vi "Main_CLIWrapper.vi"(11 "Inputs":string[](array[string])) -> (2 "Output/Failure":string, 3 "CLI Process Return Code":i32)   [LabVIEW 2019]
uses:
  <vilib>/Utility/error.llb/DialogType.ctl
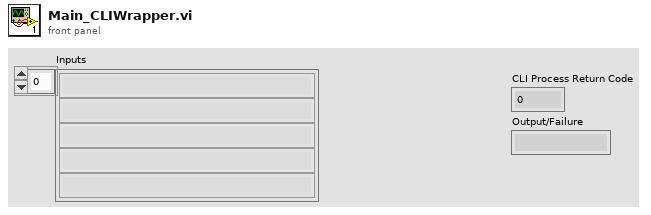
[diagram p1: front panel]
types:
  T1 = typedef "DialogType.ctl" = u16
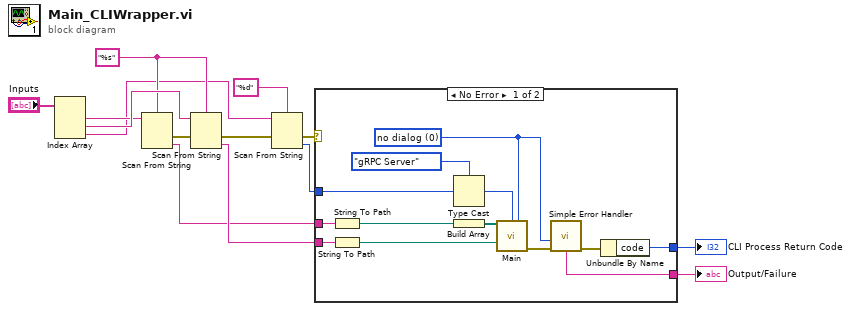
[diagram p0: block diagram]
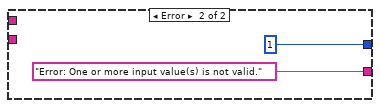
[diagram p2: hidden frame]
diagram:
  w12 = "%s" ("format string")
  n1 = Index Array "Index Array"(array="Inputs") -> (element #1=w8:string, element #2=w13:string, element #3=w4:string)  [unwired: 3 in]
  n2 = Scan From String(format string=w12, input string=w8) -> (error out=w9:errorcluster, output 1=w10:string)  [unwired: 3 in, 2 out]
  n3 = Scan From String(format string=w12, input string=w13, error in=w9) -> (error out=w3:errorcluster, output 1=w11:string)  [unwired: 2 in, 2 out]
  n4 = Scan From String(format string="%d", input string=w4, error in=w3) -> (error out=w2:errorcluster, output 1=w1:i32)  [unwired: 2 in, 2 out]
  n5 = case shown="No Error" w2 {
    tunnel: [w19 1] -> w6
    tunnel: [w16 "Error: One or more input value(s) is not valid."] -> w7
    tunnel: w11 -> [w24 _]
    tunnel: w10 -> [w27 _]
    tunnel: w1 -> [w21 _]
    frame No Error {
      w15 = T1 0 items=["no dialog", "OK message", "continue or stop message", "OK message + warnings", "continue/stop + warnings"] ("type of dialog (OK msg:1)")
      n6 = String To Path(string=w27) -> (path=w26:path)
      n7 = String To Path(string=w24) -> (path=w23:path)
      n8 = Type Cast(type=enum16{"gRPC Server", "gRPC Client", "Both"}."gRPC Server" ("Generate"), x=w21) -> (*(type *) &x=w20:enum16{"gRPC Server", "gRPC Client", "Both"})
      n9 = Build Array(w26) -> (w25:path[])
      n10 = call <vilib>:"Main.vi"("Proto File Path"=w25, "Generate"=w20, "type of dialog (OK msg:1)"=w15, "Target Project"=w23) -> ("error out"=w18:errorcluster)  [unwired: 11 in]
      n11 = call <vilib>:"Simple Error Handler.vi"("type of dialog (OK msg:1)"=w15, "error in (no error)"=w18) -> ("error out"=w17:errorcluster, "message"=w16:string)  [unwired: 3 in, 3 out]
      n12 = Unbundle By Name(w17) -> ("code"=w19:i32)
    }
    frame Error {
    }
  }
  "CLI Process Return Code" <- w6
  "Output/Failure" <- w7
